vi "Select Monitored Signal.vi"(10 "Plant Feedback":T1, 11 "Step Config":T2) -> (1 "valid":bool, 2 "target":dbl, 3 "measured":dbl)   [LabVIEW 2026]
doc: "Maps a step's monitored_io to the matching Plant Feedback signal and its setpoint from the Step Config. AI_Pressure_PT101 gives pressure_bar and pressure_sp_bar, AI_Flow_FT102 gives flow_lpm and flow_sp_lpm, AI_Displacement_LVDT103 gives displacement_mm and displacement_sp_mm. Any other monitored_io answers valid FALSE with measured and target 0. Pure function, no error terminals, AF-free."
uses:
  Typedefs/Step Config.ctl
  Typedefs/Plant Feedback.ctl
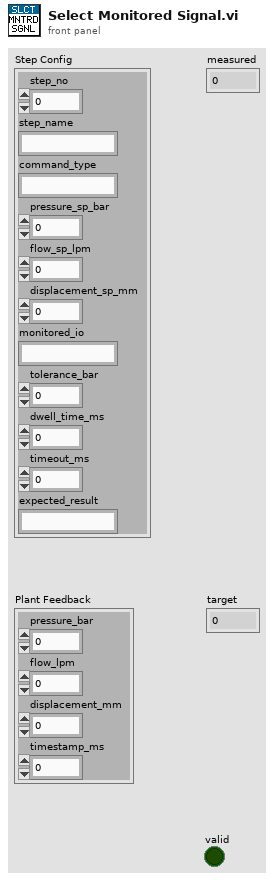
[diagram p1: front panel]
types:
  T1 = typedef "Plant Feedback.ctl" = cluster{"pressure_bar":dbl, "flow_lpm":dbl, "displacement_mm":dbl, "timestamp_ms":dbl}
  T2 = typedef "Step Config.ctl" = cluster{"step_no":i32, "step_name":string, "command_type":string, "pressure_sp_bar":dbl, "flow_sp_lpm":dbl, "displacement_sp_mm":dbl, "monitored_io":string, "tolerance_bar":dbl, "dwell_time_ms":i32, "timeout_ms":i32, "expected_result":string}
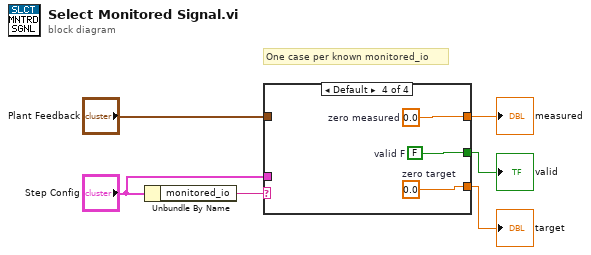
[diagram p0: block diagram]
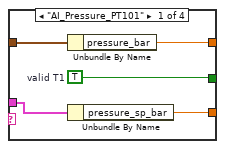
[diagram p2: hidden frame]
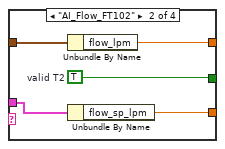
[diagram p3: hidden frame]
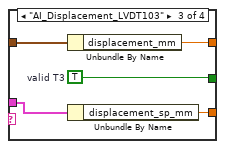
[diagram p4: hidden frame]
diagram:
  # "One case per known monitored_io"
  n1 = Unbundle By Name("Step Config") -> ("monitored_io"=w4:string)
  n2 = case shown="Default" w4 {
    tunnel: "Step Config" -> [w11 w16 w21 _]
    tunnel: "Plant Feedback" -> [w10 w15 w20 _]
    tunnel: [w9 w14 w19 w24] -> w3
    tunnel: [w8 w13 w18 w23] -> w2
    tunnel: [w7 w12 w17 w22] -> w1
    frame "AI_Pressure_PT101" {
      w7 = TRUE  # valid T1
      n3 = Unbundle By Name(w10) -> ("pressure_bar"=w9:dbl)
      n4 = Unbundle By Name(w11) -> ("pressure_sp_bar"=w8:dbl)
    }
    frame "AI_Flow_FT102" {
      w12 = TRUE  # valid T2
      n5 = Unbundle By Name(w15) -> ("flow_lpm"=w14:dbl)
      n6 = Unbundle By Name(w16) -> ("flow_sp_lpm"=w13:dbl)
    }
    frame "AI_Displacement_LVDT103" {
      w17 = TRUE  # valid T3
      n7 = Unbundle By Name(w20) -> ("displacement_mm"=w19:dbl)
      n8 = Unbundle By Name(w21) -> ("displacement_sp_mm"=w18:dbl)
    }
    frame Default {
      w22 = FALSE  # valid F
      w23 = 0.0  # zero target
      w24 = 0.0  # zero measured
    }
  }
  "measured" <- w3
  "target" <- w2
  "valid" <- w1
